vi "GetText.vi"(8 "error in":errorcluster, 11 "H1 Hydraulic":refnum<class "H1 Hydraulic.lvclass">) -> (0 "error out":errorcluster, 1 "additional text":string, 2 "text":string, 3 "H1 Hydraulic out":refnum<class "H1 Hydraulic.lvclass">, 4 "glyph":string)   [LabVIEW 2025, in "H1 Plotter.lvlib" / "H1 Hydraulic.lvclass"]
doc: "Returns the text representation of the node used for the tree control.Copyright 2017 National Instruments Corporation\n\nLicensed under the Apache License, Version 2.0 (the \"License\"); you may not use this file except in compliance with the License. You may obtain a copy of the License at http://www.apache.org/licenses/LICENSE-2.0\nUnless required by applicable law or agreed to in writing, software distributed under the License is distributed on an \"AS IS\" BASIS, WITHOUT WARRANTIES OR CONDITIONS OF ANY KIND, either express or implied. See the License for the specific language governing permissions and limitations under the License."
uses:
  H1 Hydraulic.lvclass
  H1 Hydraulic.lvclass/H1 Hydraulic.ctl
  Users/Public/Documents/Sandia National Labs/TSS Plugin/Tests/XY Plotter.lvlibp/XY  Plotter/XY Plotter.lvclass
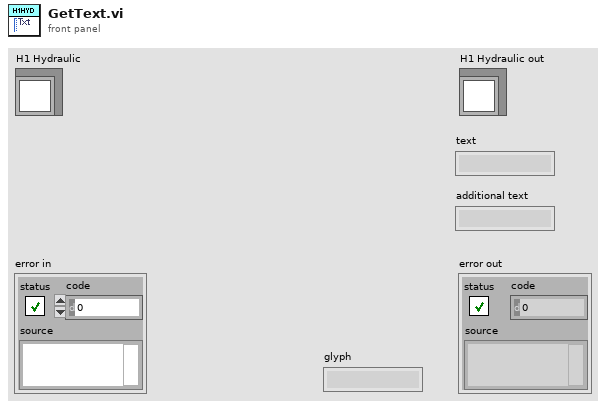
[diagram p1: front panel]
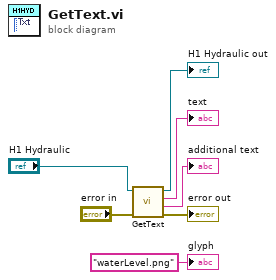
[diagram p0: block diagram]
diagram:
  n1 = call-parent "GetText.vi"("error in"="error in", "CEF_Serialize node in"="H1 Hydraulic") -> ("error out"=→"error out":errorcluster, "additional text"=→"additional text":string, "text"=→"text":string, "CEF_Serialize node out"=→"H1 Hydraulic out":refnum<class "H1 Hydraulic.lvclass">)  [unwired: 5 in, 1 out]
  "glyph" <- "waterLevel.png" ("glyph")
